vi "Patten Name Extract.vi"(8 "error in":errorcluster, 11 "Digipat source file":path) -> (0 "error out":errorcluster, 3 "pattern name":string)   [LabVIEW 2025, in "Digital Pattern Sequencer.lvclass"]
doc: "Runs DigitalPatternCompiler decompile using a temp output file based on source file name, extracts pattern name, then deletes the temp file."
uses:
  Digital Pattern Sequencer.lvclass
  Digital Pattern Sequencer.lvclass/Digital Pattern Sequencer.ctl
  <vilib>/regexp/Match Regular Expression.xnode
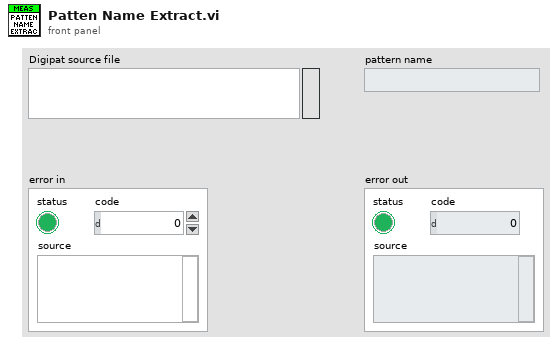
[diagram p1: front panel]
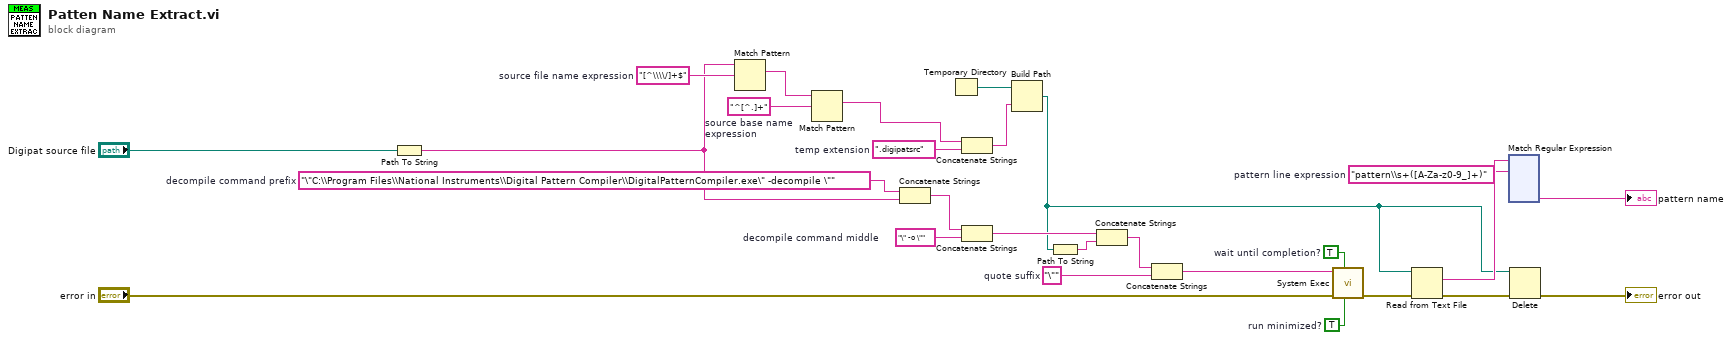
[diagram p0: block diagram]
diagram:
  w10 = "pattern\\s+([A-Za-z0-9_]+)"  # pattern line expression
  w13 = TRUE  # run minimized?
  w14 = TRUE  # wait until completion?
  w16 = "\""  # quote suffix
  w19 = "\" -o \""  # decompile command middle
  w22 = "\"C:\\Program Files\\National Instruments\\Digital Pattern Compiler\\DigitalPatternCompiler.exe\" -decompile \""  # decompile command prefix
  w23 = ".digipatsrc"  # temp extension
  w24 = "^[^.]+"  # source base name expression
  w26 = "[^\\\\/]+$"  # source file name expression
  n1 = Path To String(path="Digipat source file") -> (string=w7:string)
  n2 = Match Pattern(string=w7, regular expression=w26) -> (match substring=w25:string)  [unwired: 1 in, 3 out]
  n3 = Match Pattern(string=w25, regular expression=w24) -> (match substring=w4:string)  [unwired: 1 in, 3 out]
  n4 = Concatenate Strings(w22, w7) -> (w20:string)
  n5 = Temporary Directory() -> (w5:path)
  n6 = Concatenate Strings(w4, w23) -> (w3:string)
  n7 = Concatenate Strings(w20, w19) -> (w18:string)
  n8 = Build Path(base path=w5, name or relative path=w3) -> (appended path=w1:path)
  n9 = Path To String(path=w1) -> (string=w2:string)
  n10 = Concatenate Strings(w18, w2) -> (w17:string)
  n11 = Concatenate Strings(w17, w16) -> (w15:string)
  n12 = call <vilib>:"System Exec.vi"("run minimized? (F)"=w13, "wait until completion? (T)"=w14, "error in (no error)"="error in", "command line"=w15) -> ("error out"=w12:errorcluster)  [unwired: 4 in, 3 out]
  n13 = Read from Text File(file (use dialog)=w1, error in=w12) -> (text=w11:string, error out=w9:errorcluster)  [unwired: 2 in, 2 out]
  n14 = xnode "Match Regular Expression"("input string"=w11, "regular expression"=w10) -> ("submatch 1"=→"pattern name":string)  [unwired: 4 in, 5 out]
  n15 = Delete(path (use dialog)=w1, error in=w9) -> (error out=→"error out":errorcluster)  [unwired: 3 in, 2 out]
